vi "CSE ISP - create example submenu.vi"(7 "menu tag":string="EXMPL", 8 "error in":errorcluster, 11 "ISP menu":refnum<k9>) -> (0 "error out":errorcluster, 3 "dup ISP menu":refnum<k9>)   [LabVIEW 2021]
doc: "::: CalcExpress Toolkit :::\nCopyright (c) 2000-2026 Konstantin Shifershteyn. All rights reserved."
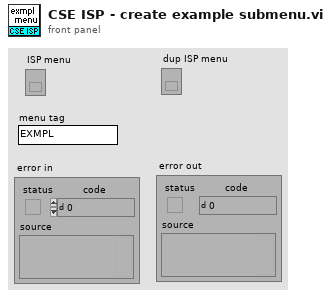
[diagram p1: front panel]
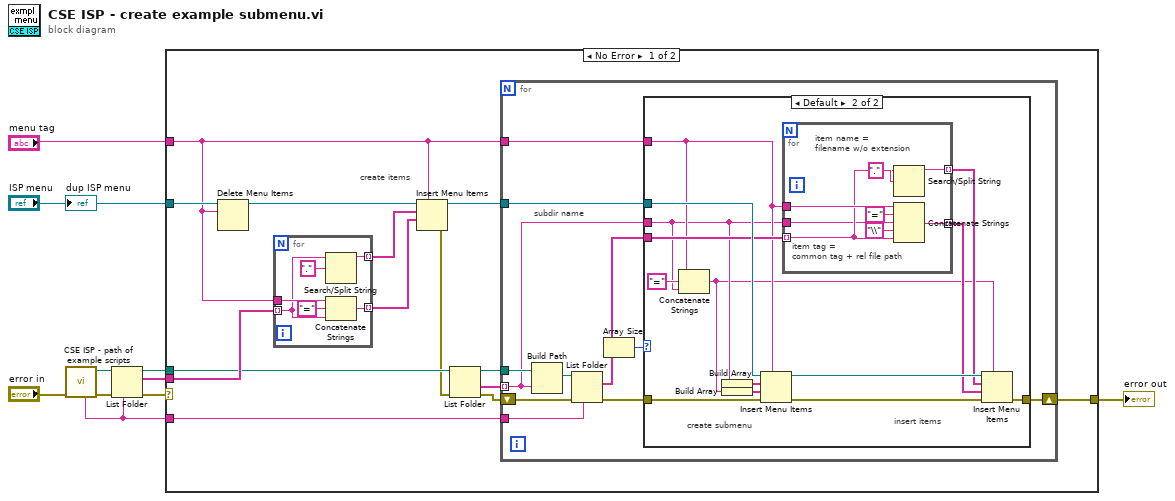
[diagram p0: block diagram]
diagram:
  n1 = call "CSE ISP - path of example scripts.vi"("error in"="error in") -> ("error out"=w1:errorcluster, "path of example scripts"=w9:path, "pattern out"=w3:string)  [unwired: 6 in, 2 out]
  n2 = List Folder(path=w9, pattern=w3, error in=w1) -> (path out=w8:path, filenames=w10:string[], error out=w4:errorcluster)  [unwired: 1 in, 1 out]
  n3 = case shown="No Error" w4 {
    selector: w4 -> [_ w65]
    tunnel: w10 -> [w24 _]
    tunnel: w3 -> [w21 _]
    tunnel: w8 -> [w17 _]
    tunnel: [w14 w65] -> w7
    tunnel: "ISP menu" -> [w13 _]
    tunnel: "menu tag" -> [w11 _]
    frame No Error {
      # "create items"
      n4 = Delete Menu Items(8:w11, 9:w13) -> (3:w12:refnum<k9>)  [unwired: 2 in, 1 out]
      n5 = for {
        tunnel: w24 -> [w63] mode=indexing
        tunnel: w11 -> [w64]
        tunnel: [w61] -> w23 mode=indexing
        tunnel: [w60] -> w22 mode=indexing
        n6 = Search/Split String(string=w63, search string/char (-)="." ("search char (-)")) -> (substring before match=w61:string)  [unwired: 1 in, 2 out]
        n7 = Concatenate Strings(w64, "=" ("menu tag"), w63) -> (w60:string)
      }
      n8 = Insert Menu Items(5:w11, 7:w22, 8:w23, 9:w12) -> (0:w16:errorcluster, 3:w20:refnum<k9>)  [unwired: 2 in, 1 out]
      n9 = List Folder(path=w17, error in=w16) -> (path out=w18:path, folder names=w19:string[], error out=w15:errorcluster)  [unwired: 2 in, 1 out]
      n10 = for {
        tunnel: w19 -> [w27] mode=indexing
        tunnel: w18 -> [w35]
        tunnel: w21 -> [w29]
        tunnel: w11 -> [w32]
        tunnel: w20 -> [w31]
        shift-right: [w25] -> w14
        shift-left: w15 -> [w28]
        # "subdir name"
        n11 = Build Path(base path=w35, name or relative path=w27) -> (appended path=w34:path)
        n12 = List Folder(path=w34, pattern=w29, error in=w28) -> (filenames=w30:string[], error out=w26:errorcluster)  [unwired: 1 in, 2 out]
        n13 = Array Size(array=w30) -> (size(s)=w33:i32)
        n14 = case shown="Default" w33 {
          tunnel: w32 -> [_ w40]
          tunnel: w31 -> [_ w50]
          tunnel: w30 -> [_ w45]
          tunnel: w27 -> [_ w38]
          tunnel: [w36 w42] -> w25
          tunnel: w26 -> [w36 w44]
          frame 0 {
          }
          frame Default {
            # "insert items"
            # "create submenu"
            n15 = Concatenate Strings(w40, "=", w38) -> (w37:string)
            n16 = Build Array(w38) -> (w46:string[])
            n17 = Build Array(w37) -> (w41:string[])
            n18 = Insert Menu Items(5:w40, 6:w44, 7:w41, 8:w46, 9:w50) -> (0:w43:errorcluster, 3:w49:refnum<k9>)  [unwired: 1 in, 1 out]
            n19 = for {
              tunnel: w40 -> [w58]
              tunnel: [w56] -> w48 mode=indexing
              tunnel: [w55] -> w47 mode=indexing
              tunnel: w45 -> [w52] mode=indexing
              tunnel: w38 -> [w51]
              # "item tag =\ncommon tag + rel file path"
              # "item name =\nfilename w/o extension"
              n20 = Search/Split String(string=w52, search string/char (-)="." ("search char (-)")) -> (substring before match=w56:string)  [unwired: 1 in, 2 out]
              n21 = Concatenate Strings(w58, "=" ("menu tag"), w51, "\\", w52) -> (w55:string)
            }
            n22 = Insert Menu Items(5:w37, 6:w43, 7:w47, 8:w48, 9:w49) -> (0:w42:errorcluster)  [unwired: 1 in, 2 out]
          }
        }
      }
    }
    frame Error {
    }
  }
  "error out" <- w7
  "dup ISP menu" <- "ISP menu"
